vi "update.name.request.vi"(8 "error in":errorcluster, 11 "Title":string) -> (0 "error out":errorcluster, 1 "Request":string)   [LabVIEW 2020, in "Run.lvclass"]
uses:
  Run.lvclass
  Run.lvclass/Run.ctl
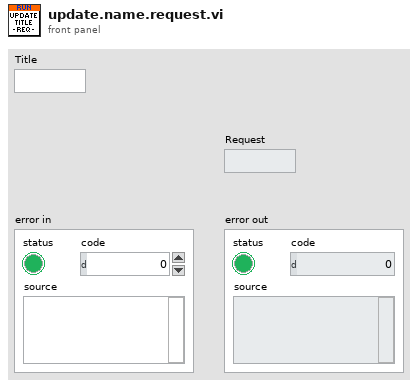
[diagram p1: front panel]
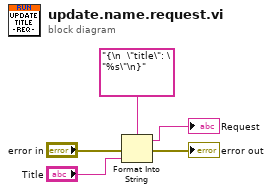
[diagram p0: block diagram]
diagram:
  n1 = Format Into String(format string="{\n  \"title\": \"%s\"\n}", error in="error in", "Title") -> (resulting string=→"Request":string, error out=→"error out":errorcluster)  [unwired: 1 in]
